vi "CopyOverlay.vi"(7 "Groups":string[](array[string]), 8 "error in":errorcluster, 10 "Dst Reference In":T1, 11 "Src Reference In":T1) -> (0 "error out":errorcluster, 3 "Dst Reference Out":T1)   [LabVIEW 2020, in "OpenLvVision_Overlays.lvlib"]
doc: "Copies an image overlay from a source to a destination image. If the destination image already contains an overlay, this VI combines the source overlay with the pre-existing one."
uses:
  OpenLvVision_Overlays.lvlib
  <vilib>/OpenLvVision/OpenLvVision_Image/Management/TypeDef/OLV Image.ctl
  <vilib>/OpenLvVision/OpenLvVision_Image/Management/OLV Management.lvlib
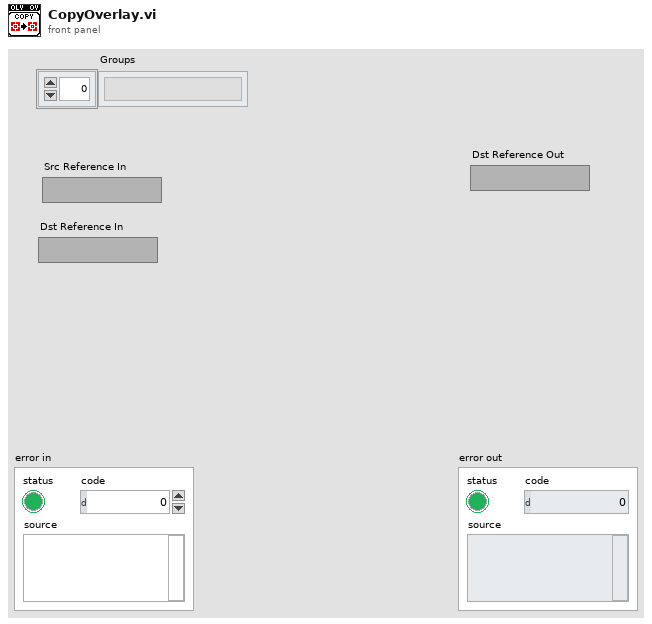
[diagram p1: front panel]
types:
  T1 = typedef "OLV OpenLvVision_Image.lvlib/OLV Management.lvlib/OLV Image.ctl" = refnum<image>
  T2 = typedef "IMAQ Image.ctl" = refnum<image>
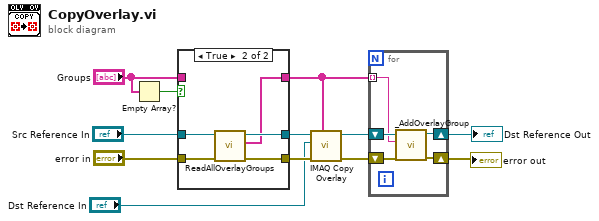
[diagram p0: block diagram]
diagram:
  n1 = Empty Array?(array="Groups") -> (empty?=w7:bool)
  n2 = case shown="True" w7 {
    tunnel: "Groups" -> [w15 _]
    tunnel: [w15 w16] -> w6
    tunnel: "error in" -> [w14 w20]
    tunnel: [w14 w18] -> w4
    tunnel: "Src Reference In" -> [w13 w19]
    tunnel: [w13 w17] -> w1
    frame False {
    }
    frame True {
      n3 = call "ReadAllOverlayGroups.vi"("error in"=w20, "Image Reference In"=w19) -> ("error out"=w18:errorcluster, "OverlayGroups"=w16:string[], "Image Reference Out"=w17:T1)  [unwired: 7 in]
    }
  }
  n4 = call "IMAQ Copy Overlay"("Groups"=w6, "error in (no error)"=w4, "Image Dst"="Dst Reference In", "Image Src"=w1) -> ("error out"=w11:errorcluster, "Image Dst Out"=w12:T2)  [unwired: 6 in]
  n5 = for {
    shift-right: [w22] -> w10
    shift-left: w11 -> [w24]
    shift-right: [w23] -> w9
    shift-left: w12 -> [w25]
    tunnel: w6 -> [w21] mode=indexing
    n6 = call "_AddOverlayGroup.vi"("error in"=w24, "GroupName"=w21, "Image Reference In"=w25) -> ("error out"=w22:errorcluster, "Image Reference Out"=w23:T1)  [unwired: 7 in]
  }
  "error out" <- w10
  "Dst Reference Out" <- w9
